vi "clone.vi"(0 "reference":refnum<class "RectangularNode.lvclass">, 5 "error in (no error)":errorcluster) -> (14 "reference out":refnum<class "RectangularNode.lvclass">, 15 "clonedRectanglularNode":refnum<class "AbstractNode.lvclass">, 19 "error out":errorcluster)   [LabVIEW 2020, in "RectangularNode.lvclass"]
doc: "public Object clone()"
uses:
  <resource>/Framework/Providers/Open_GDS/UML/RectangularNode_class/RectangularNode.lvclass
  C:/Program Files (x86)/National Instruments/LabVIEW 2020/resource/Framework/Providers/Open_GDS/UML/AbstractNode_class/AbstractNode.lvclass
  <resource>/Framework/Providers/Open_GDS/UML/AbstractNode_class/AbstractNode.lvclass
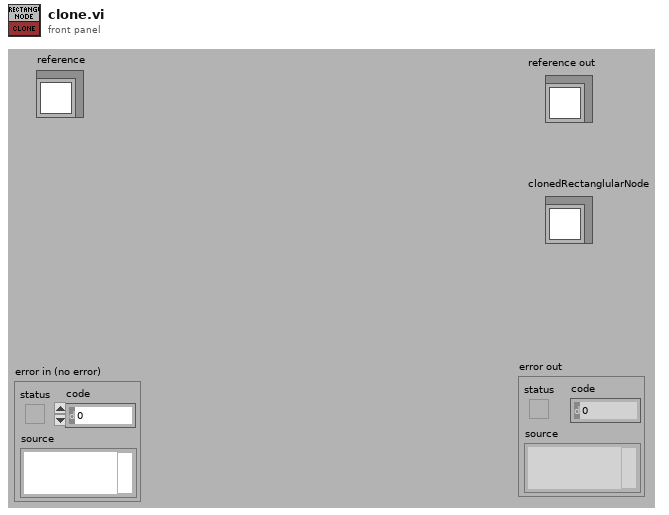
[diagram p1: front panel]
types:
  T1 = typedef "RectangularNode.lvclass/ObjectAttributes.ctl" = cluster{"bounds":T2}
  T2 = typedef "Rectangle Rectangle2D.ctl" = cluster{"x":dbl, "y":dbl, "width":dbl, "height":dbl}
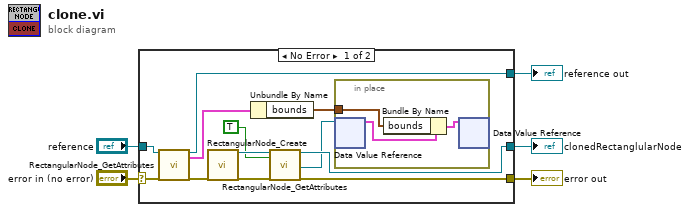
[diagram p0: block diagram]
diagram:
  n1 = case shown="No Error" "error in (no error)" {
    selector: "error in (no error)" -> [w15 w21]
    tunnel: "reference" -> [w17 w22]
    tunnel: [w16 w21] -> w4
    tunnel: [w10 w22] -> w3
    tunnel: [w14 _] -> w1
    frame No Error {
      n2 = call <resource>:"RectangularNode_GetAttributes.vi"("reference in"=w17, "error in (no error)"=w15) -> ("reference out"=w10:refnum<class "RectangularNode.lvclass">, "Data"=w8:T1, "error out"=w11:errorcluster)  [unwired: 1 in, 14 out]
      n3 = call <resource>:"RectangularNode_Create.vi"("error in (no error)"=w11) -> ("reference out"=w13:refnum<class "RectangularNode.lvclass">, "error out"=w12:errorcluster)  [unwired: 17 in]
      n4 = Unbundle By Name(w8) -> ("bounds"=w6:T2)
      n5 = call <resource>:"RectangularNode_GetAttributes.vi"("reference in"=w13, "OnlyGetDvrReference(False)"=TRUE, "error in (no error)"=w12) -> ("reference out"=w14:refnum<class "RectangularNode.lvclass">, "DataRef"=w7:refnum<data-value>, "error out"=w16:errorcluster)  [unwired: 13 in, 1 out]
      n6 = in-place {
        in-place-border: w6 -> [w19]
        n7 = in-place-dvr #1(w7) -> (w20:T1)  [unwired: 1 out]
        n8 = Bundle By Name(cluster=w20, "bounds"=w19) -> (w18:T1)
        n9 = in-place-dvr #1(w18) -> ()  [unwired: 2 out]
      }
    }
    frame Error {
    }
  }
  "reference out" <- w3
  "error out" <- w4
  "clonedRectanglularNode" <- w1
